vi "N4_401.vi"(4 "error in":T15, 7 "Command":T16) -> (0 "error out":T15, 3 "Response":T13)   [LabVIEW 2018]
uses:
  MOKO_LabViewLibrary/MokoLowLevel/MokoLowLovelControl/MLLC_Command.ctl
  MOKO_LabViewLibrary/MokoLowLevel/MokoLowLovelControl/MLLC_Error.ctl
  MOKO_LabViewLibrary/MokoLowLevel/MokoLowLovelControl/MLLC_Mode.ctl
  MOKO_LabViewLibrary/MokoLowLevel/MokoLowLovelControl/MLLC_Response.ctl
  MOKO_LabViewLibrary/MokoLowLevel/MokoLowLovelControl/MLLC_DriverName.ctl
  MOKO_LabViewLibrary/MokoLowLevel/MokoLowLovelControl/MLLC_Request.ctl
  MOKO_LabViewLibrary/MokoLowLevel/MokoLowLovelControl/MLLC_ErrorCode.ctl
  MOKO_LabViewLibrary/MokoLowLevel/MokoLowLovelControl/MLLC_ResponseInit.ctl
  MOKO_LabViewLibrary/MokoLowLevel/MokoLowLovelControl/MLLC_ConnectCluster.ctl
  MOKO_LabViewLibrary/MokoLowLevel/MokoLowLovelControl/MLLC_InterfaceType.ctl
  MOKO_LabViewLibrary/MokoLowLevel/MokoLowLovelControl/MLLC_OpenedSession.ctl
  MOKO_LabViewLibrary/MokoLowLevel/MokoLowLovelControl/MLLC_InterfaceSettings.ctl
  MOKO_LabViewLibrary/MokoLowLevel/MokoLowLovelControl/MLLC_InterfaceKind.ctl
  MOKO_LabViewLibrary/MokoLowLevel/MokoLowLovelControl/MLLC_Boolean.ctl
  MOKO_LabViewLibrary/MokoLowLevel/MokoLowLovelControl/MLLC_Delay.ctl
panel:
  in  "Settings":T8={"Saved Data"=variant, "Data"={"Connect"={"InterfaceType"=enum."VISA", "OpenedSession"="COM1", "InterfaceSettings"={"Interface"=enum."RS232", "EOS 4 read"=enum."LF (\\n)", "EOS 4 write"=enum."LF (\\n)", "TMO, ms"=10000, "Sett"=variant(cluster{"Baud Rate":u32, "Data Bits":u16, "Parity":u16, "Stop Bits":u16, "Flow Control":u16, "Eho":bool} {"Baud Rate"=75, "Data Bits"=0, "Parity"=0, "Stop Bits"=0, "Flow Control"=0, "Eho"=FALSE})}}, "RangeAuto"=TRUE, "SwitchOFF"=TRUE, "Range"=0.0}}
  in  "ResponseInit":T9="N4-"
  in  "Error Code":T10=5470
  in  "Request":T11="IDN?"
  in  "Driver Name":T12="N4_X01"
  in  "Mode":T14=enum."Check"
  # "Í4-X01"
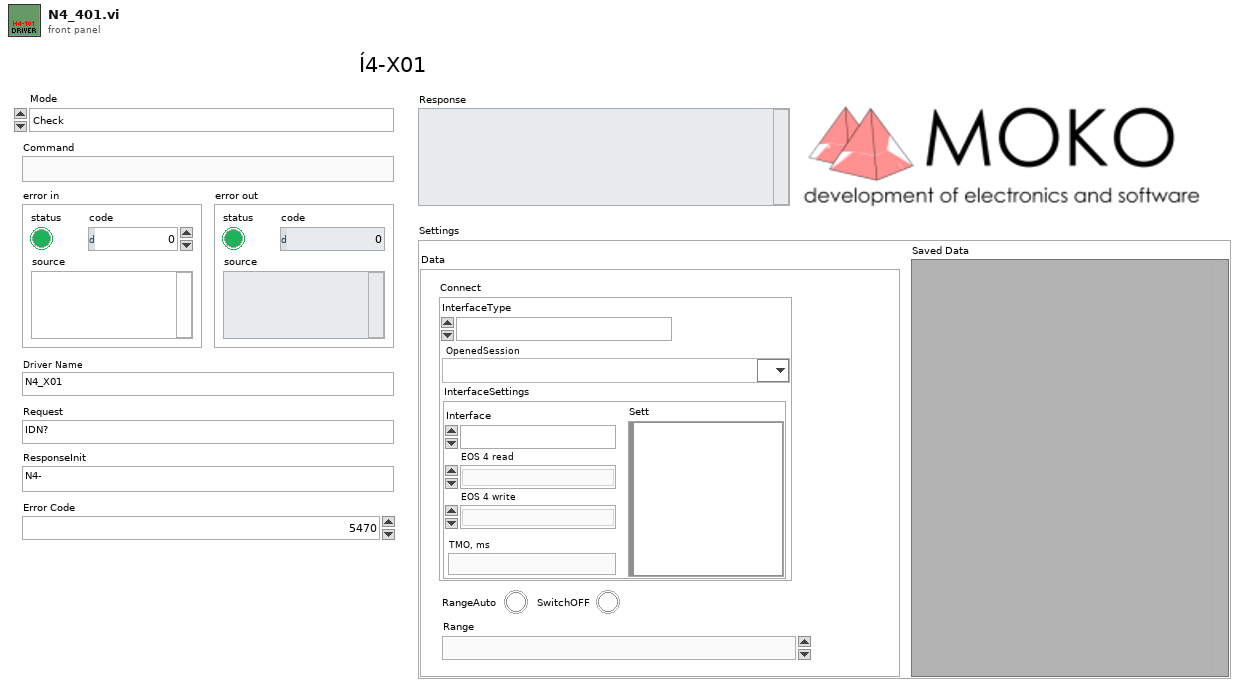
[diagram p1: front panel]
types:
  T1 = typedef "MLLC_ConnectCluster.ctl" = cluster{"InterfaceType":T2, "OpenedSession":T3, "InterfaceSettings":T4}
  T2 = typedef "MLLC_InterfaceType.ctl" = enum16{"VISA", "Prologix USB-GPIB"}
  T3 = typedef "MLLC_OpenedSession.ctl" = refnum<visa-resource-name>
  T4 = typedef "MLLC_InterfaceSettings.ctl" = cluster{"Interface":T5, "EOS 4 read":enum16{"Default (=EOS 4 write)", "CR (\\r)", "LF (\\n)", "None"}, "EOS 4 write":enum16{"CR+LF (\\r\\n)", "CR (\\r)", "LF (\\n)", "None"}, "TMO, ms":i32, "Sett":variant}
  T5 = typedef "MLLC_InterfaceKind.ctl" = enum16{"RS232", "GPIB", "USB", "Ethernet", "another"}
  T6 = typedef "MLLC_Boolean.ctl" = bool
  T7 = typedef "MLLC_Delay.ctl" = dbl
  T8 = cluster{"Saved Data":variant, "Data":cluster{"Connect":T1, "RangeAuto":T6, "SwitchOFF":T6, "Range":T7}}
  T9 = typedef "MLLC_ResponseInit.ctl" = string
  T10 = typedef "MLLC_ErrorCode.ctl" = u32
  T11 = typedef "MLLC_Request.ctl" = string
  T12 = typedef "MLLC_DriverName.ctl" = string
  T13 = typedef "MLLC_Response.ctl" = string
  T14 = typedef "MLLC_Mode.ctl" = enum16{"get", "set", "close", "Init", "Check"}
  T15 = typedef "MLLC_Error.ctl" = errorcluster
  T16 = typedef "MLLC_Command.ctl" = string
  T17 = cluster{"Connect":T1, "RangeAuto":T6, "SwitchOFF":T6, "Range":T7}
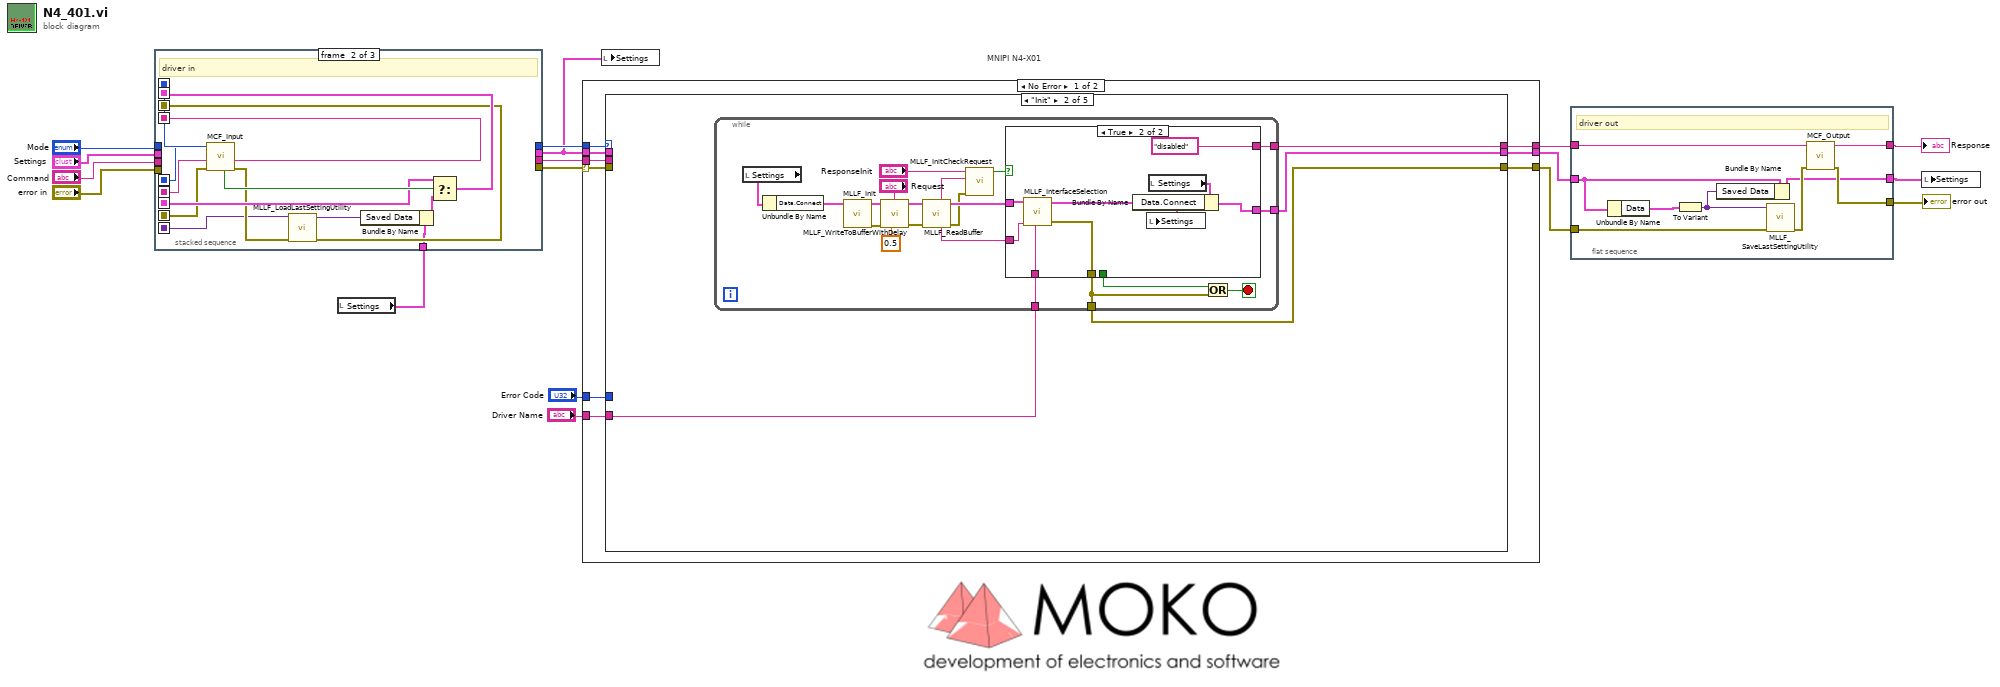
[diagram p0: block diagram]
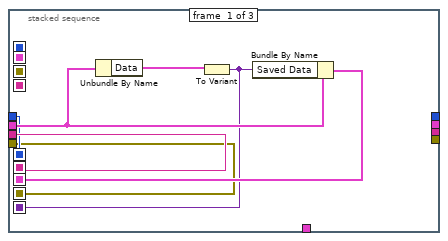
[diagram p2: hidden frame]
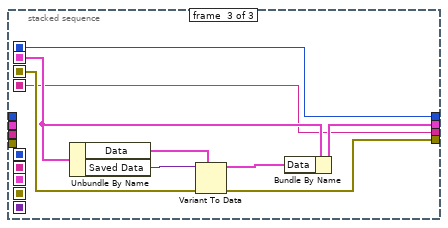
[diagram p3: hidden frame]
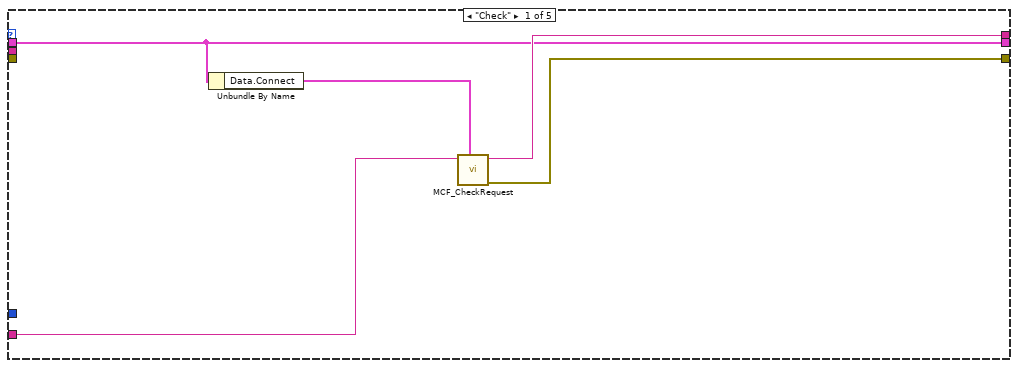
[diagram p4: hidden frame]
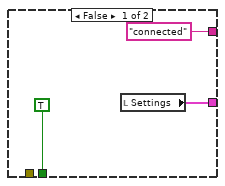
[diagram p5: hidden frame]
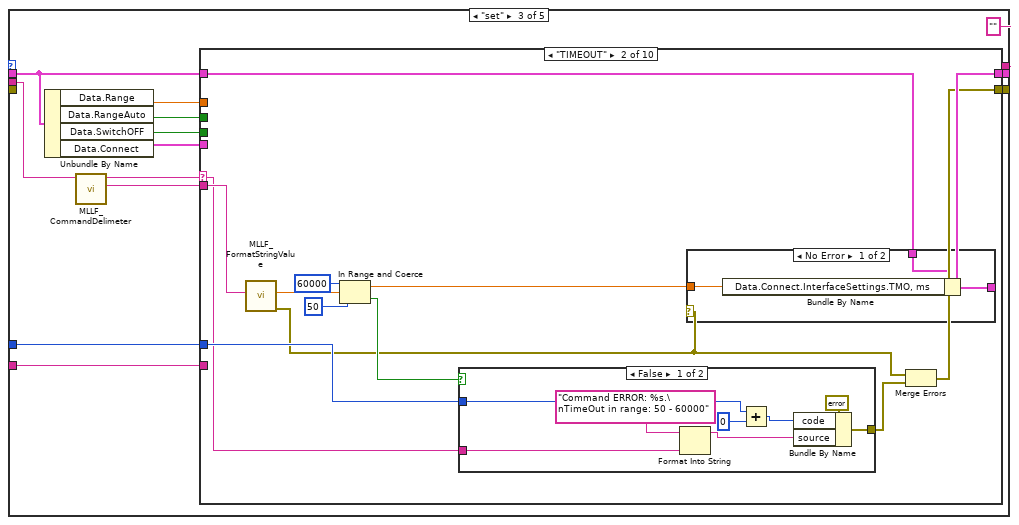
[diagram p6: hidden frame]
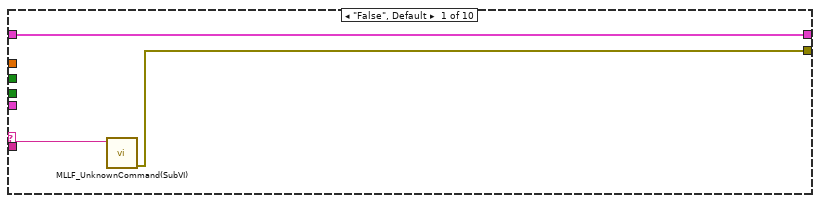
[diagram p7: hidden frame]
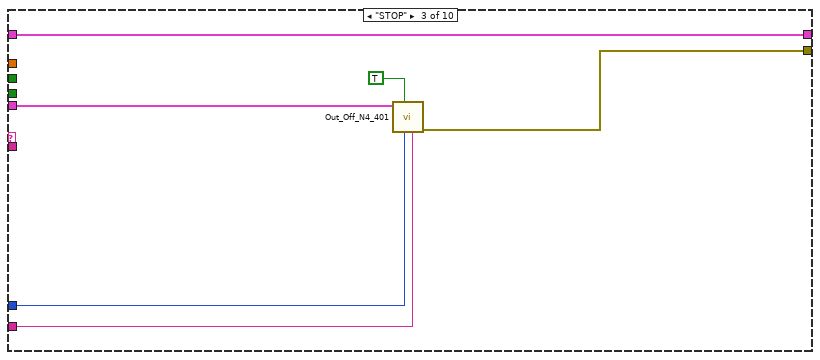
[diagram p10: hidden frame]
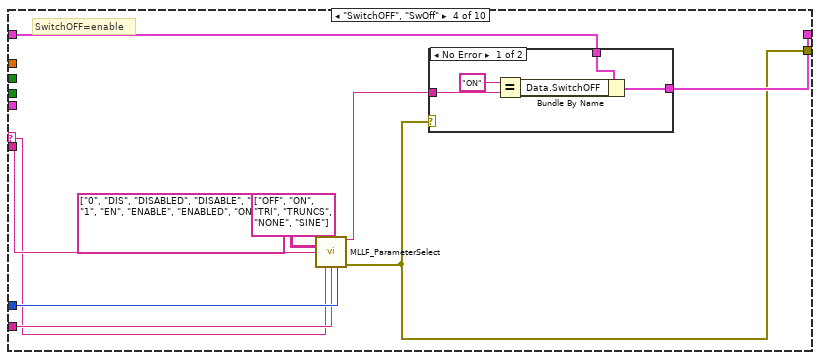
[diagram p11: hidden frame]
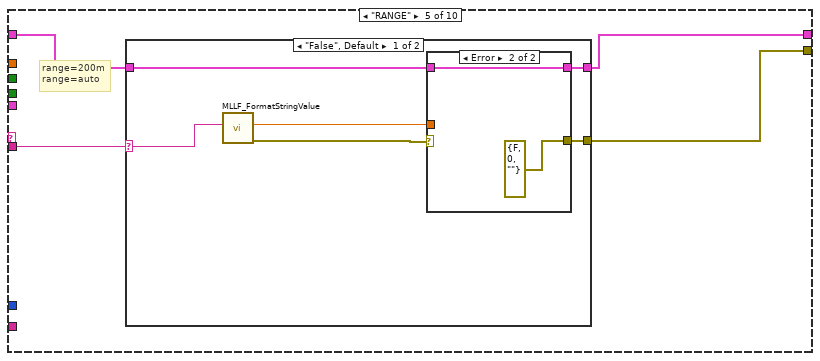
[diagram p13: hidden frame]
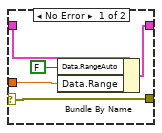
[diagram p14: hidden frame]
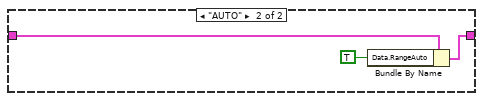
[diagram p15: hidden frame]
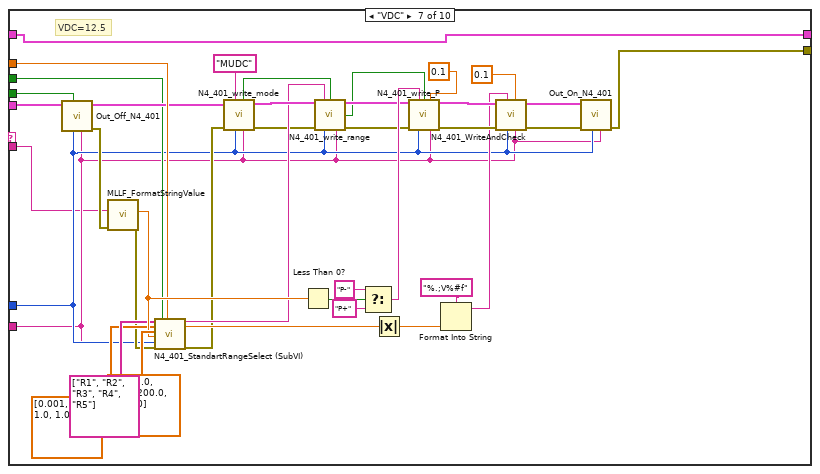
[diagram p17: hidden frame]
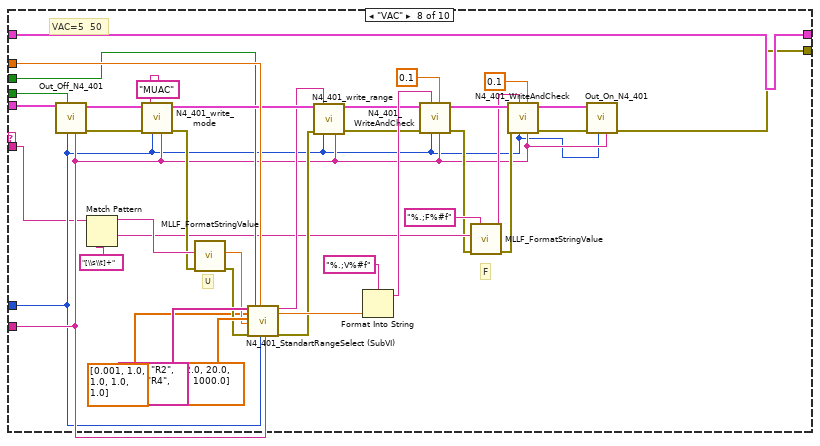
[diagram p18: hidden frame]
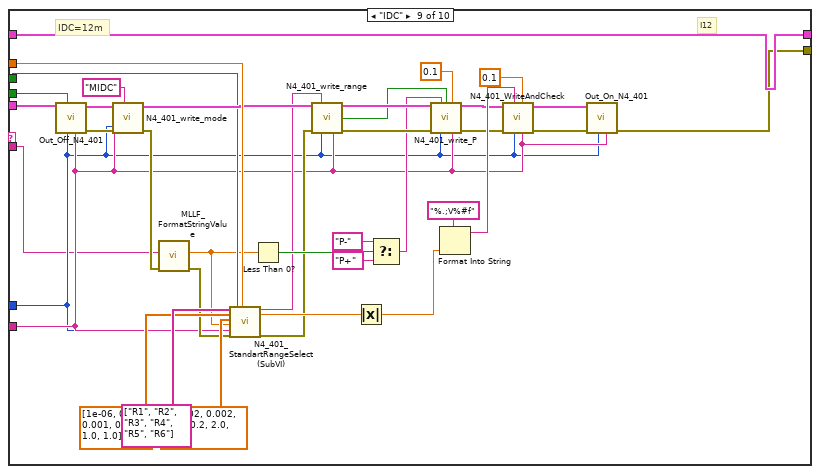
[diagram p19: hidden frame]
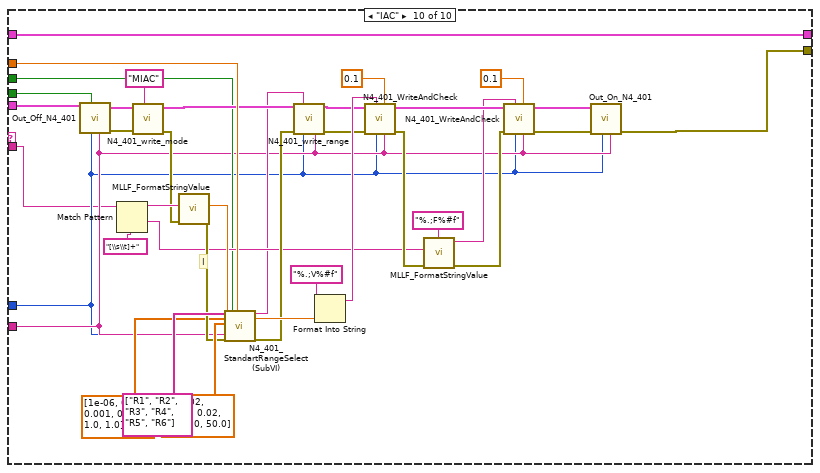
[diagram p20: hidden frame]
diagram:
  # "MNIPI N4-X01"
  n1 = local read "Settings"() -> (w7:T8)
  n2 = stacked-sequence {
    seq-local: [w20 _ _] -> [_ w36 _]
    seq-local: [w19 _ _] -> [_ w37 _]
    seq-local: [w22 _ _] -> [_ w32 _]
    seq-local: [w18 _ _] -> [_ w31 _]
    seq-local: [w21 _ _] -> [_ w27 _]
    seq-local: [_ w28 _] -> [_ _ w44]
    seq-local: [_ w38 _] -> [_ _ w41]
    seq-local: [_ w35 _] -> [_ _ w40]
    seq-local: [_ w34 _] -> [_ _ w45]
    tunnel: "Command" -> [w20 _ _]
    tunnel: "Mode" -> [w19 _ _]
    tunnel: "error in" -> [w18 _ _]
    tunnel: "Settings" -> [w23 _ _]
    tunnel: w7 -> [_ w26 _]
    tunnel: [_ _ w40] -> w9
    tunnel: [_ _ w43] -> w10
    tunnel: [_ _ w42] -> w8
    tunnel: [_ _ w41] -> w11
    frame #0 {
      n3 = Unbundle By Name(w23) -> ("Data"=w24:T17)
      n4 = To Variant(anything=w24) -> (Variant=w21:variant)
      n5 = Bundle By Name(cluster=w23, "Saved Data"=w21) -> (w22:T8)
    }
    frame #1 {
      # "driver in"
      n6 = call "MCF_Input.vi"("Error In"=w31, "Command in"=w36, "Mode in"=w37) -> ("Error Out"=w30:errorcluster, "Command out"=w35:string, "Mode out"=w38:T14, "Boolean"=w33:bool)  [unwired: 5 in]
      n7 = call "MLLF_LoadLastSettingUtility.vi"("Error In"=w30, "Save data in"=w27) -> ("Error Out"=w28:errorcluster, "Save data out"=w25:variant)  [unwired: 8 in]
      n8 = Bundle By Name(cluster=w26, "Saved Data"=w25) -> (w29:T8)
      n9 = Select(t=w32, s=w33, f=w29) -> (s? t:f=w34:T8)
    }
    frame #2 {
      n10 = Unbundle By Name(w45) -> ("Data"=w46:T17, "Saved Data"=w39:variant)
      n11 = Variant To Data(error in=w44, type=w46, Variant=w39) -> (data=w47:T17, error out=w42:errorcluster)
      n12 = Bundle By Name(cluster=w45, "Data"=w47) -> (w43:T8)
    }
  }
  n13 = case shown="No Error" w8 {
    selector: w8 -> [w52 w372]
    tunnel: [w54 w372] -> w4
    tunnel: w11 -> [w56 _]
    tunnel: [w55 "" ("String")] -> w6
    tunnel: w9 -> [w53 _]
    tunnel: w10 -> [w49 w371]
    tunnel: "Error Code" -> [w51 _]
    tunnel: "Driver Name" -> [w50 _]
    tunnel: [w48 w371] -> w5
    frame No Error {
      n14 = case shown="\"Init\"" w56 {
        tunnel: [w60 w65 "" ("String") w334 "" ("String")] -> w55
        tunnel: [w61 w63 w98 w333 w368] -> w54
        tunnel: w53 -> [_ _ w108 w344 _]
        tunnel: w52 -> [_ _ _ _ _]
        tunnel: w51 -> [_ _ w107 w341 _]
        tunnel: w50 -> [w59 w62 w104 w340 _]
        tunnel: w49 -> [w58 _ w106 w343 w367]
        tunnel: [w58 w64 w105 w342 w367] -> w48
        frame "Check" {
          n15 = Unbundle By Name(w58) -> ("Data.Connect"=w57:T1)
          n16 = call "MCF_CheckRequest.vi"("Permanent data.Connect"=w57, "Driver Name"=w59) -> ("Error Out"=w61:errorcluster, "Output String"=w60:string)  [unwired: 8 in]
        }
        frame "Init" {
          n17 = while {
            tunnel: [w77] -> w63
            tunnel: [w69] -> w64
            tunnel: [w68] -> w65
            tunnel: w62 -> [w67]
            stop <- w75 stop-if-true
            n18 = local read "Settings"() -> (w84:T8)
            n19 = Unbundle By Name(w84) -> ("Data.Connect"=w78:T1)
            n20 = call "MLLF_Init.vi"("DriverConnect in"=w78) -> ("Error Out"=w80:errorcluster, "DriverConnect out"=w79:T1)  [unwired: 7 in]
            n21 = call "MLLF_WriteToBufferWithDelay.vi"("Delay Time ( 0,05 s)"=0.5 ("Delay Time (s)"), "Command"="Request", "Error In"=w80, "DriverConnect in"=w79) -> ("Error Out"=w73:errorcluster, "DriverConnect out"=w82:T1)  [unwired: 6 in]
            n22 = call "MLLF_ReadBuffer.vi"("Error In"=w73, "DriverConnect in"=w82) -> ("Error Out"=w71:errorcluster, "DriverConnect out"=w81:T1, "String"=w66:string)  [unwired: 6 in]
            n23 = call "MLLF_InitCheckRequest.vi"("error in (no error)"=w71, "Answer"=w66, "Response Init"="ResponseInit") -> ("Design"=w70:bool)  [unwired: 5 in, 3 out]
            n24 = case shown="True" w70 {
              tunnel: w81 -> [_ w94]
              tunnel: [_ w95] -> w77
              tunnel: [TRUE _] -> w76
              tunnel: [w85 w91] -> w69
              tunnel: ["connected" "disabled"] -> w68
              tunnel: w67 -> [_ w89]
              tunnel: w66 -> [_ w88]
              frame False {
                n25 = local read "Settings"() -> (w85:T8)
              }
              frame True {
                n26 = call "MLLF_InterfaceSelection.vi"("Driver Name"=w89, "Answer:"=w88, "DriverConnect in"=w94) -> ("error out"=w95:T15, "DriverConnect out"=w93:T1)  [unwired: 4 in, 3 out]
                n27 = local read "Settings"() -> (w92:T8)
                n28 = Bundle By Name(cluster=w92, "Data.Connect"=w93) -> (w91:T8)
                n29 = local write "Settings"(w91) -> ()
              }
            }
            n30 = Or(x=w76, y=w77) -> (x .or. y?=w75:bool)
          }
        }
        frame "set" {
          n31 = Unbundle By Name(w106) -> ("Data.Range"=w99:T7, "Data.RangeAuto"=w100:T6, "Data.SwitchOFF"=w101:T6, "Data.Connect"=w102:T1)
          n32 = call "MLLF_CommandDelimeter.vi"("command with param"=w108) -> ("param 1"=w96:string, "command"=w97:string)  [unwired: 6 in, 3 out]
          n33 = case shown="\"TIMEOUT\"" w97 {
            selector: w97 -> [w110 w112 _ w143 _ _ _ _ _ _]
            tunnel: w96 -> [_ w115 _ w144 w162 _ w180 w220 w257 w296]
            tunnel: [w109 w118 w141 w147 w161 _ w181 w219 w258 w295] -> w98
            tunnel: w107 -> [_ w119 w139 w146 _ _ w184 w221 w260 w297]
            tunnel: w106 -> [w111 w123 w142 w149 w160 w179 w218 w255 w293 w331]
            tunnel: [w111 w124 w142 w148 w159 w179 w218 w255 w293 w331] -> w105
            tunnel: w102 -> [_ _ w138 _ _ _ w202 w256 w294 w332]
            tunnel: w104 -> [_ _ w140 w145 _ _ w183 w222 w261 w298]
            tunnel: w101 -> [_ _ _ _ _ _ w201 w247 w288 w322]
            tunnel: w100 -> [_ _ _ _ _ _ w195 w233 w268 w303]
            tunnel: w99 -> [_ _ _ _ _ _ w203 w239 w280 w314]
            frame "False", Default {
              n34 = call "MLLF_UnknownCommand(SubVI).vi"("Unknown command"=w110) -> ("error out"=w109:errorcluster)  [unwired: 10 in]
            }
            frame "TIMEOUT" {
              n35 = call "MLLF_FormatStringValue.vi"("String Value"=w115) -> ("error out"=w113:T15, "number"=w114:dbl)  [unwired: 8 in, 1 out]
              n36 = In Range and Coerce(upper limit=60000, x=w114, lower limit=50) -> (coerced(x)=w120:dbl, In Range?=w116:bool)
              n37 = case shown="False" w116 {
                tunnel: [w131 _] -> w117
                tunnel: w119 -> [w130 _]
                tunnel: w112 -> [w129 _]
                frame False {
                  n38 = Format Into String(format string="Command ERROR: %s.\nTimeOut in range: 50 - 60000", w129) -> (resulting string=w133:string)  [unwired: 2 in, 1 out]
                  n39 = Add(x=w130, y=0) -> (x+y=w134:T10)
                  n40 = Bundle By Name(cluster=errorcluster {"status"=TRUE, "code"=0, "source"=""} ("error out"), "code"=w134, "source"=w133) -> (w131:errorcluster)
                }
                frame True {
                }
              }
              n41 = case shown="No Error" w113 {
                tunnel: [w127 w128] -> w124
                tunnel: w123 -> [w126 w128]
                tunnel: w120 -> [w125 _]
                frame No Error {
                  n42 = Bundle By Name(cluster=w126, "Data.Connect.InterfaceSettings.TMO, ms"=w125) -> (w127:T8)
                }
                frame Error {
                }
              }
              n43 = Merge Errors(w113, w117) -> (w118:errorcluster)
            }
            frame "STOP" {
              n44 = call "Out_Off_N4_401.vi"("Driver Name"=w140, "Error Code"=w139, "SwitchOFF"=TRUE, "DriverConnect in"=w138) -> ("error out"=w141:T15)  [unwired: 6 in, 1 out]
            }
            frame "SwitchOFF", "SwOff" {
              # "SwitchOFF=enable"
              n45 = call "MLLF_ParameterSelect.vi"("Command to equipment"=string[] ["OFF", "ON", "TRI", "TRUNCS", "NONE", "SINE"] ("Parameters"), "Names"=string[][] [["0", "DIS", "DISABLED", "DISABLE", "OFF"], ["1", "EN", "ENABLE", "ENABLED", "ON"]], "Input"=w144, "Command"=w143, "Driver Name"=w145, "Error Code"=w146) -> ("Choice"=w152:string, "Error Out"=w147:errorcluster)  [unwired: 8 in]
              n46 = case shown="No Error" w147 {
                tunnel: w152 -> [w157 _]
                tunnel: w149 -> [w155 w158]
                tunnel: [w154 w158] -> w148
                frame No Error {
                  n47 = Equal?(x="ON", y=w157) -> (x = y?=w153:bool)
                  n48 = Bundle By Name(cluster=w155, "Data.SwitchOFF"=w153) -> (w154:T8)
                }
                frame Error {
                }
              }
            }
            frame "RANGE" {
              # "range=200m\nrange=auto"
              n49 = case shown="\"False\", Default" w162 {
                selector: w162 -> [w168 _]
                tunnel: [w163 _] -> w161
                tunnel: [w166 w178] -> w159
                tunnel: w160 -> [w167 w177]
                frame "False", Default {
                  n50 = call "MLLF_FormatStringValue.vi"("String Value"=w168) -> ("error out"=w164:T15, "number"=w165:dbl)  [unwired: 8 in, 1 out]
                  n51 = case shown="Error" w164 {
                    selector: w164 -> [w169 _]
                    tunnel: w167 -> [w172 w175]
                    tunnel: [w171 w175] -> w166
                    tunnel: w165 -> [w170 _]
                    tunnel: [w169 errorcluster {"status"=FALSE, "code"=0, "source"=""} ("error IO")] -> w163
                    frame No Error {
                      n52 = Bundle By Name(cluster=w172, "Data.RangeAuto"=FALSE ("RangeAuto"), "Data.Range"=w170) -> (w171:T8)
                    }
                    frame Error {
                    }
                  }
                }
                frame "AUTO" {
                  n53 = Bundle By Name(cluster=w177, "Data.RangeAuto"=TRUE ("RangeAuto")) -> (w178:T8)
                }
              }
            }
            frame "<----MAIN FUNCTIONS---->" {
            }
            frame "VDC" {
              # "VDC=12.5"
              n54 = call "Out_Off_N4_401.vi"("Driver Name"=w183, "Error Code"=w184, "SwitchOFF"=w201, "DriverConnect in"=w202) -> ("error out"=w191:T15, "DriverConnect out"=w197:T1)  [unwired: 6 in]
              n55 = call "MLLF_FormatStringValue.vi"("error in"=w191, "String Value"=w180) -> ("error out"=w193:T15, "number"=w216:dbl)  [unwired: 7 in, 1 out]
              n56 = call "N4_401_StandartRangeSelect (SubVI).vi"("Range Command"=string[] ["R1", "R2", "R3", "R4", "R5"] ("RangeCommand"), "Scale Array"=dbl[] [0.001, 1.0, 1.0, 1.0, 1.0] ("ScaleArray"), "Range Digit"=dbl[] [0.2, 2.0, 20.0, 200.0, 1000.0] ("RangeDigit"), "Control Point"=w216, "Error In"=w193, "RangeAuto"=w195, "Range"=w203, "Error Code"=w184, "Driver Name"=w183) -> ("Range Out"=w196:string, "Scaled value"=w214:dbl, "Error Out"=w190:errorcluster)  [unwired: 8 in]
              n57 = call "N4_401_write_mode.vi"("Driver Name"=w183, "Error Code"=w184, "Command"="MUDC" ("String"), "error in"=w190, "DriverConnect in"=w197) -> ("error out"=w189:T15, "DriverConnect out"=w200:T1, "ModeWasChacged"=w188:T6)  [unwired: 4 in]
              n58 = Less Than 0?(x=w216) -> (x < 0?=w213:bool)
              n59 = call "N4_401_write_range.vi"("DriverConnect in"=w200, "Command range"=w196, "ModeIsChanged?"=w188, "error in"=w189, "Error Code"=w184, "Driver Name"=w183) -> ("DriverConnect out"=w199:T1, "RangeWasChanged"=w192:T6, "error out"=w198:T15)  [unwired: 7 in]
              n60 = Select(t="P-" ("String"), s=w213, f="P+" ("String")) -> (s? t:f=w210:string)
              n61 = Absolute Value(x=w214) -> (abs(x)=w207:dbl)
              n62 = call "N4_401_write_P.vi"("DriverConnect in"=w199, "P"=w210, "RangeIsChanged?"=w192, "Command Time (s)"=0.1, "error in"=w198, "Error Code"=w184, "Driver Name"=w183) -> ("DriverConnect out"=w208:T1, "error out"=w209:T15)  [unwired: 7 in]
              n63 = Format Into String(format string="%.;V%#f", w207) -> (resulting string=w205:string)  [unwired: 2 in, 1 out]
              n64 = call "N4_401_WriteAndCheck.vi"("Driver Name"=w183, "Command Time (s)"=0.1, "Error Code"=w184, "Command"=w205, "error in"=w209, "DriverConnect in"=w208) -> ("error out"=w185:T15, "DriverConnect out"=w186:T1)  [unwired: 4 in]
              n65 = call "Out_On_N4_401.vi"("Driver Name"=w183, "Error Code"=w184, "error in"=w185, "DriverConnect in"=w186) -> ("error out"=w181:T15)  [unwired: 6 in, 1 out]
            }
            frame "VAC" {
              # "VAC=5  50"
              # "F"
              # "U"
              n66 = call "Out_Off_N4_401.vi"("Driver Name"=w222, "Error Code"=w221, "SwitchOFF"=w247, "DriverConnect in"=w256) -> ("error out"=w232:T15, "DriverConnect out"=w238:T1)  [unwired: 6 in]
              n67 = Match Pattern(string=w220, regular expression="[\\s\\t]+") -> (before substring=w240:string, after substring=w229:string)  [unwired: 1 in, 2 out]
              n68 = call "N4_401_write_mode.vi"("Driver Name"=w222, "Error Code"=w221, "Command"="MUAC" ("String"), "error in"=w232, "DriverConnect in"=w238) -> ("error out"=w231:T15, "DriverConnect out"=w237:T1)  [unwired: 4 in, 1 out]
              n69 = call "MLLF_FormatStringValue.vi"("error in"=w231, "String Value"=w240) -> ("error out"=w249:T15, "number"=w250:dbl)  [unwired: 7 in, 1 out]
              n70 = call "N4_401_StandartRangeSelect (SubVI).vi"("Range Command"=string[] ["R1", "R2", "R3", "R4", "R5"] ("RangeCommand"), "Scale Array"=dbl[] [0.001, 1.0, 1.0, 1.0, 1.0] ("ScaleArray"), "Range Digit"=dbl[] [0.2, 2.0, 20.0, 200.0, 1000.0] ("RangeDigit"), "Control Point"=w250, "Error In"=w249, "RangeAuto"=w233, "Range"=w239, "Error Code"=w221, "Driver Name"=w222) -> ("Range Out"=w236:string, "Scaled value"=w244:dbl, "Error Out"=w230:errorcluster)  [unwired: 8 in]
              n71 = call "N4_401_write_range.vi"("DriverConnect in"=w237, "Command range"=w236, "error in"=w230, "Error Code"=w221, "Driver Name"=w222) -> ("DriverConnect out"=w235:T1, "error out"=w234:T15)  [unwired: 8 in, 1 out]
              n72 = Format Into String(format string="%.;V%#f", w244) -> (resulting string=w241:string)  [unwired: 2 in, 1 out]
              n73 = call "N4_401_WriteAndCheck.vi"("Driver Name"=w222, "Command Time (s)"=0.1, "Error Code"=w221, "Command"=w241, "error in"=w234, "DriverConnect in"=w235) -> ("error out"=w228:T15, "DriverConnect out"=w246:T1)  [unwired: 4 in]
              n74 = call "MLLF_FormatStringValue.vi"("error in"=w228, "String Value"=w229, "Format"="%.;F%#f" ("format string")) -> ("error out"=w245:T15, "String Value Formated"=w242:T16)  [unwired: 6 in, 1 out]
              n75 = call "N4_401_WriteAndCheck.vi"("Driver Name"=w222, "Command Time (s)"=0.1, "Error Code"=w221, "Command"=w242, "error in"=w245, "DriverConnect in"=w246) -> ("error out"=w223:T15, "DriverConnect out"=w224:T1)  [unwired: 4 in]
              n76 = call "Out_On_N4_401.vi"("Driver Name"=w222, "Error Code"=w221, "error in"=w223, "DriverConnect in"=w224) -> ("error out"=w219:T15)  [unwired: 6 in, 1 out]
            }
            frame "IDC" {
              # "IDC=12m"
              # "I12"
              n77 = call "Out_Off_N4_401.vi"("Driver Name"=w261, "Error Code"=w260, "SwitchOFF"=w288, "DriverConnect in"=w294) -> ("error out"=w272:T15, "DriverConnect out"=w274:T1)  [unwired: 6 in]
              n78 = call "N4_401_write_mode.vi"("Driver Name"=w261, "Error Code"=w260, "Command"="MIDC" ("String"), "error in"=w272, "DriverConnect in"=w274) -> ("error out"=w271:T15, "DriverConnect out"=w277:T1)  [unwired: 4 in, 1 out]
              n79 = call "MLLF_FormatStringValue.vi"("error in"=w271, "String Value"=w257) -> ("error out"=w287:T15, "number"=w265:dbl)  [unwired: 7 in, 1 out]
              n80 = call "N4_401_StandartRangeSelect (SubVI).vi"("Range Command"=string[] ["R1", "R2", "R3", "R4", "R5", "R6"] ("RangeCommand"), "Scale Array"=dbl[] [1e-06, 0.001, 0.001, 0.001, 1.0, 1.0] ("ScaleArray"), "Range Digit"=dbl[] [0.0002, 0.002, 0.02, 0.2, 2.0, 50.0] ("RangeDigit"), "Control Point"=w265, "Error In"=w287, "RangeAuto"=w268, "Range"=w280, "Error Code"=w260, "Driver Name"=w261) -> ("Range Out"=w273:string, "Scaled value"=w289:dbl, "Error Out"=w270:errorcluster)  [unwired: 8 in]
              n81 = Less Than 0?(x=w265) -> (x < 0?=w284:bool)
              n82 = call "N4_401_write_range.vi"("DriverConnect in"=w277, "Command range"=w273, "error in"=w270, "Error Code"=w260, "Driver Name"=w261) -> ("DriverConnect out"=w278:T1, "RangeWasChanged"=w266:T6, "error out"=w279:T15)  [unwired: 8 in]
              n83 = Absolute Value(x=w289) -> (abs(x)=w281:dbl)
              n84 = Select(t="P-" ("String"), s=w284, f="P+" ("String")) -> (s? t:f=w269:string)
              n85 = call "N4_401_write_P.vi"("DriverConnect in"=w278, "P"=w269, "RangeIsChanged?"=w266, "Command Time (s)"=0.1, "error in"=w279, "Error Code"=w260, "Driver Name"=w261) -> ("DriverConnect out"=w276:T1, "error out"=w275:T15)  [unwired: 7 in]
              n86 = Format Into String(format string="%.;V%#f", w281) -> (resulting string=w283:string)  [unwired: 2 in, 1 out]
              n87 = call "N4_401_WriteAndCheck.vi"("Driver Name"=w261, "Command Time (s)"=0.1, "Error Code"=w260, "Command"=w283, "error in"=w275, "DriverConnect in"=w276) -> ("error out"=w262:T15, "DriverConnect out"=w263:T1)  [unwired: 4 in]
              n88 = call "Out_On_N4_401.vi"("Driver Name"=w261, "Error Code"=w260, "error in"=w262, "DriverConnect in"=w263) -> ("error out"=w258:T15)  [unwired: 6 in, 1 out]
            }
            frame "IAC" {
              # "I"
              n89 = call "Out_Off_N4_401.vi"("Driver Name"=w298, "Error Code"=w297, "SwitchOFF"=w322, "DriverConnect in"=w332) -> ("error out"=w308:T15, "DriverConnect out"=w310:T1)  [unwired: 6 in]
              n90 = Match Pattern(string=w296, regular expression="[\\s\\t]+") -> (before substring=w329:string, after substring=w305:string)  [unwired: 1 in, 2 out]
              n91 = call "N4_401_write_mode.vi"("Command"="MIAC" ("String"), "error in"=w308, "DriverConnect in"=w310) -> ("error out"=w307:T15, "DriverConnect out"=w313:T1)  [unwired: 6 in, 1 out]
              n92 = call "MLLF_FormatStringValue.vi"("error in"=w307, "String Value"=w329) -> ("error out"=w325:T15, "number"=w324:dbl)  [unwired: 7 in, 1 out]
              n93 = call "N4_401_StandartRangeSelect (SubVI).vi"("Range Command"=string[] ["R1", "R2", "R3", "R4", "R5", "R6"] ("RangeCommand"), "Scale Array"=dbl[] [1e-06, 0.001, 0.001, 0.001, 1.0, 1.0] ("ScaleArray"), "Range Digit"=dbl[] [0.0002, 0.002, 0.02, 0.2, 2.0, 50.0] ("RangeDigit"), "Control Point"=w324, "Error In"=w325, "RangeAuto"=w303, "Range"=w314, "Error Code"=w297, "Driver Name"=w298) -> ("Range Out"=w304:string, "Scaled value"=w317:dbl, "Error Out"=w306:errorcluster)  [unwired: 8 in]
              n94 = call "N4_401_write_range.vi"("DriverConnect in"=w313, "Command range"=w304, "error in"=w306, "Error Code"=w297, "Driver Name"=w298) -> ("DriverConnect out"=w312:T1, "error out"=w311:T15)  [unwired: 8 in, 1 out]
              n95 = Format Into String(format string="%.;V%#f", w317) -> (resulting string=w321:string)  [unwired: 2 in, 1 out]
              n96 = call "N4_401_WriteAndCheck.vi"("Driver Name"=w298, "Command Time (s)"=0.1, "Error Code"=w297, "Command"=w321, "error in"=w311, "DriverConnect in"=w312) -> ("error out"=w316:T15, "DriverConnect out"=w320:T1)  [unwired: 4 in]
              n97 = call "MLLF_FormatStringValue.vi"("error in"=w316, "String Value"=w305, "Format"="%.;F%#f" ("format string")) -> ("error out"=w315:T15, "String Value Formated"=w319:T16)  [unwired: 6 in, 1 out]
              n98 = call "N4_401_WriteAndCheck.vi"("Driver Name"=w298, "Command Time (s)"=0.1, "Error Code"=w297, "Command"=w319, "error in"=w315, "DriverConnect in"=w320) -> ("error out"=w299:T15, "DriverConnect out"=w300:T1)  [unwired: 4 in]
              n99 = call "Out_On_N4_401.vi"("Driver Name"=w298, "Error Code"=w297, "error in"=w299, "DriverConnect in"=w300) -> ("error out"=w295:T15)  [unwired: 6 in, 1 out]
            }
          }
        }
        frame "get" {
          n100 = Unbundle By Name(w343) -> ("Data.Connect"=w337:T1)
          n101 = call "MLLF_CommandDelimeter.vi"("command with param"=w344) -> ("param 1"=w335:string, "command"=w336:string)  [unwired: 6 in, 3 out]
          n102 = case shown="\"AMPL\", \"AMPLITUDE\"" w336 {
            selector: w336 -> [w346 _ _]
            tunnel: w335 -> [_ _ _]
            tunnel: [w345 _ w354] -> w339
            tunnel: w341 -> [_ _ _]
            tunnel: [w349 w352 w365] -> w342
            tunnel: w343 -> [w349 w352 w365]
            tunnel: [w347 w350 w364] -> w338
            tunnel: w337 -> [_ _ w357]
            tunnel: w340 -> [_ _ _]
            frame "False", Default {
              n103 = call "MLLF_UnknownCommand(SubVI).vi"("Unknown command"=w346) -> ("error out"=w345:errorcluster)  [unwired: 10 in]
              n104 = Build Array(0 ("TimeOut")) -> (w347:i32[])
            }
            frame "TIMEOUT" {
              n105 = Unbundle By Name(w352) -> ("Data.Connect.InterfaceSettings.TMO, ms"=w351:i32)
              n106 = Build Array(w351) -> (w350:i32[])
            }
            frame "AMPL", "AMPLITUDE" {
              n107 = call "MLLF_WriteToBuffer.vi"("String"="V?" ("Error Query"), "DriverConnect in"=w357) -> ("error out"=w362:T15, "DriverConnect out"=w358:T1)  [unwired: 6 in]
              n108 = call "500ms12"("error in (no error)"=w362, "Delay Time (s)"=0.5) -> ("error out"=w363:errorcluster)  [unwired: 9 in]
              n109 = call "MLLF_ReadBuffer.vi"("Error In"=w363, "DriverConnect in"=w358) -> ("Error Out"=w355:errorcluster, "String"=w360:string)  [unwired: 6 in, 1 out]
              n110 = call "MLLF_FormatStringValue.vi"("error in"=w355, "String Value"=w360, "Format"="%#e" ("format string")) -> ("error out"=w354:T15, "number"=w356:dbl)  [unwired: 6 in, 1 out]
              n111 = Build Array(w356) -> (w364:dbl[])
            }
          }
          n112 = call "MLLF_FormatOutputValueWithUnits.vi"("error in"=w339, "ValuesIn"=w338) -> ("error out"=w333:T15, "Result string"=w334:T16)  [unwired: 8 in]
        }
        frame "close" {
          n113 = Unbundle By Name(w367) -> ("Data.Connect.OpenedSession"=w369:T3)
          n114 = VISA Close(VISA resource name=w369) -> (error out=w368:errorcluster)  [unwired: 1 in]
        }
      }
    }
    frame Error {
    }
  }
  n115 = local write "Settings"(w10) -> ()
  n116 = flat-sequence {
    tunnel: [w381] -> w1
    tunnel: [w380] -> w3
    tunnel: w6 -> [w379]
    tunnel: w4 -> [w378]
    tunnel: w5 -> [w374]
    tunnel: [w376] -> w2
    frame #0 {
      # "driver out"
      n117 = Unbundle By Name(w374) -> ("Data"=w373:T17)
      n118 = To Variant(anything=w373) -> (Variant=w375:variant)
      n119 = Bundle By Name(cluster=w374, "Saved Data"=w375) -> (w376:T8)
      n120 = call "MLLF_SaveLastSettingUtility.vi"("error in"=w378, "Saved Data"=w375) -> ("error out"=w377:T15)  [unwired: 8 in, 1 out]
      n121 = call "MCF_Output.vi"("Error In"=w377, "Input"=w379) -> ("Error Out"=w380:errorcluster, "Output"=w381:string)  [unwired: 8 in]
    }
  }
  n122 = local write "Settings"(w2) -> ()
  "error out" <- w3
  "Response" <- w1
